vi "check Event Status Bit for OPC.vi"(8 "error in (no error)":errorcluster, 11 "FSV-40N in":refnum<class "FSV-40N.lvclass">) -> (0 "error out":errorcluster, 2 "OPC Bit Changed?":bool, 3 "FSV-40N out":refnum<class "FSV-40N.lvclass">)   [LabVIEW 2023, in "Spectrum Analyzer.lvlib" / "FSV-40N.lvclass"]
uses:
  FSV-40N.lvclass
  FSV-40N.lvclass/FSV-40N.ctl
  Spectrum Analyzer.lvlib
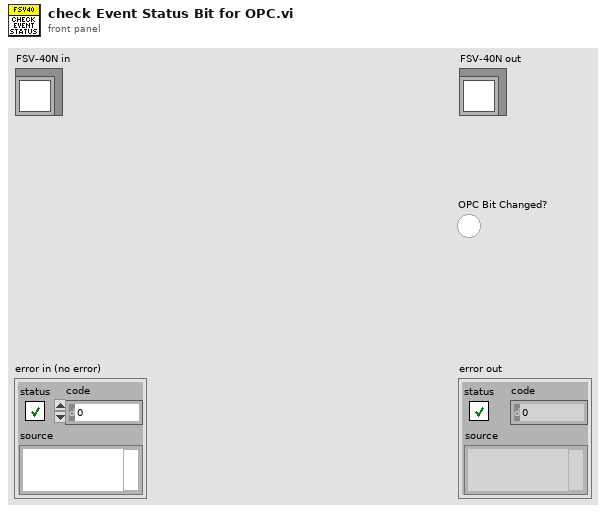
[diagram p1: front panel]
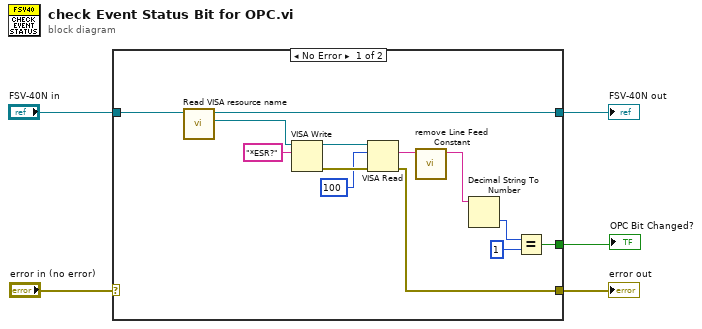
[diagram p0: block diagram]
diagram:
  n1 = case shown="No Error" "error in (no error)" {
    selector: "error in (no error)" -> [_ w20]
    tunnel: "FSV-40N in" -> [w18 w19]
    tunnel: [w7 w20] -> w3
    tunnel: [w10 w19] -> w2
    tunnel: [w6 _] -> w1
    frame No Error {
      n2 = call "Read VISA resource name.vi"("FSV-40N in"=w18) -> ("VISA resource name"=w11:refnum<visa-resource-name>, "FSV-40N out"=w10:refnum<class "FSV-40N.lvclass">)  [unwired: 8 in, 1 out]
      n3 = VISA Write(VISA resource name=w11, write buffer="*ESR?") -> (VISA resource name out=w17:refnum<visa-resource-name>, error out=w16:errorcluster)  [unwired: 1 in, 1 out]
      n4 = VISA Read(VISA resource name=w17, byte count=u32 100, error in (no error)=w16) -> (read buffer=w9:string, error out=w7:errorcluster)  [unwired: 2 out]
      n5 = call "remove Line Feed Constant.vi"("Input String"=w9) -> ("Line Feed Removed String"=w8:string)  [unwired: 10 in]
      n6 = Decimal String To Number(string=w8) -> (number=w13:i32)  [unwired: 2 in, 1 out]
      n7 = Equal?(x=w13, y=1) -> (x = y?=w6:bool)
    }
    frame Error {
    }
  }
  "error out" <- w3
  "FSV-40N out" <- w2
  "OPC Bit Changed?" <- w1
